vi "Modbus Comm Tester.vi"() -> ()   [LabVIEW 2012]
doc: "Modbus Comm Tester\n\nThis VI demonstrates the usage of the Modbus Master API for both TCP and Serial connections.\nIt is also a useful tool for testing communication with your modbus device. You can test different\ncommunication parameters and coil/register address ranges without having to write any code.\n\nCopyright (c) 2016, Plasmionique Inc.\nAll rights reserved.\n\nLicense: BSD (2-Clause) - http://opensource.org/licenses/BSD-2-Clause"
uses:
  MB_PDU/MB_ReadDevID Codes.ctl
  MB_Master/MB_Master.lvclass
  MB_ADU/MB_ADU.lvclass/MB_ADU.ctl
  MB_ADU/Read TX Data.vi
  MB_ADU/Read RX Data.vi
  MB_ADU/Read RX Timestamp.vi
  MB_Master_Serial/MB_Master_Serial.lvclass
  MB Master.lvlib
  MB_Master_TCP/MB_Master_TCP.lvclass
  MB_ADU/MB_ADU.lvclass
panel:
  in  "Device ID code":T1=1 items=["Basic"=1, "Regular"=2, "Extended"=3, "Single"=4]
  in  "object ID":u8 caption="Object ID"
  in  "Read ID":bool
  out "Open?":bool caption="Connected"
  in  "Tab Control 2":enum32{"Comm Settings", "Comm Status"}(tab)
  in  "Open":bool
  in  "Close":bool
  in  "Type":enum16{"Serial", "TCP"}(ring) caption="Connection Type"
  in  "Tab Control":enum32{"Page 1", "Page 2"}(tab)
  in  "Retries":i32=1
  in  "Timeout (ms)":u32=300
  in  "Flow Control":u16(ring) items=["None", "XON/XOFF", "RTS/CTS", "XON/XOFF & RTS/CTS", "DTR/DSR", "XON/XOFF & DTR/DSR"]
  in  "Parity":u16(ring) items=["None", "Odd", "Even", "Mark", "Space"]
  in  "Stop Bits":u16(ring)=10 items=["1.0"=10, "1.5"=15, "2.0"=20]
  in  "Baud Rate (bps)":u32(ring)=19200 items=["9600"=9600, "19200"=19200, "38400"=38400, "57600"=57600, "115200"=115200, "460800"=460800, "921600"=921600]
  in  "Slave Address":u8=1
  in  "Mode":enum16{"RTU", "ASCII"}(ring)
  in  "COM Port":refnum<visa-resource-name>
  in  "TCP_Port":u16=502 caption="Port"
  in  "IP Address":string="localhost"
  in  "TCP_Timeout":i32=10000 caption="Timeout (ms)"
  in  "TCP_Slave ID":u8=255 caption="Slave ID" format="%.0x"
  in  "Poll Period (ms)":i32=100
  out "Last Error Status":errorcluster
  out "Last RX":string
  out "Last TX":string
  out "Last RX Time":string
  out "Last Error Time":string
  out "dt (ms)":u32
  out "ID objects":string[](array[string]) caption="ID Objects"
  in  "coil Poll":bool
  in  "HR Poll":bool
  in  "DI Poll":bool
  in  "IR Poll":bool
  in  "Write Hld Regs":bool
  in  "Read Hld Regs":bool
  in  "HR QTY":u16=1 caption="Quantity"
  in  "HR SA":u16 caption="Starting Address"
  in  "Holding Registers":u16[](array[numeric])
  in  "Read In Regs":bool
  in  "IR QTY":u16=1 caption="Quantity"
  in  "IR SA":u16 caption="Starting Address"
  out "Input Registers":u16[](array[numeric])
  in  "Read DIs":bool
  in  "DI QTY":u16=1 caption="Quantity"
  in  "DI SA":u16 caption="Starting Address"
  out "Discrete Inputs":bool[](array[boolean])
  in  "Write Coils":bool
  in  "Read Coils":bool
  in  "Coil QTY":u16=1 caption="Quantity"
  in  "Coil SA":u16 caption="Starting Address"
  in  "Coils":bool[](array[boolean])
  # "Input Registers"
  # "Discrete Inputs"
  # "Device ID Objects"
  # "Holding Registers"
  # "Coils"
  # "Communication Settngs"
  # "Communication Status"
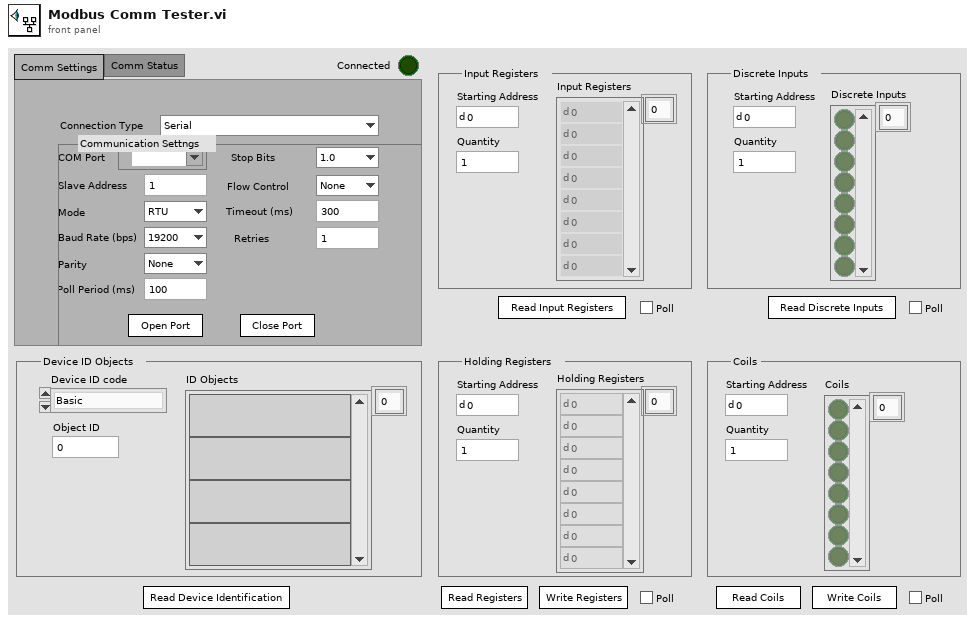
[diagram p1: front panel]
types:
  T1 = typedef "MB Master.lvlib/MB_ReadDevID Codes.ctl" = u8
  T2 = cluster{"baud rate (bps)":u32, "stop bits":u16, "parity":u16, "flow control":u16, "timeout":u32, "retries":i32}
  T3 = typedef "MB Master.lvlib/MB_DevID Object.ctl" = cluster{"ID":u8, "Value":string}
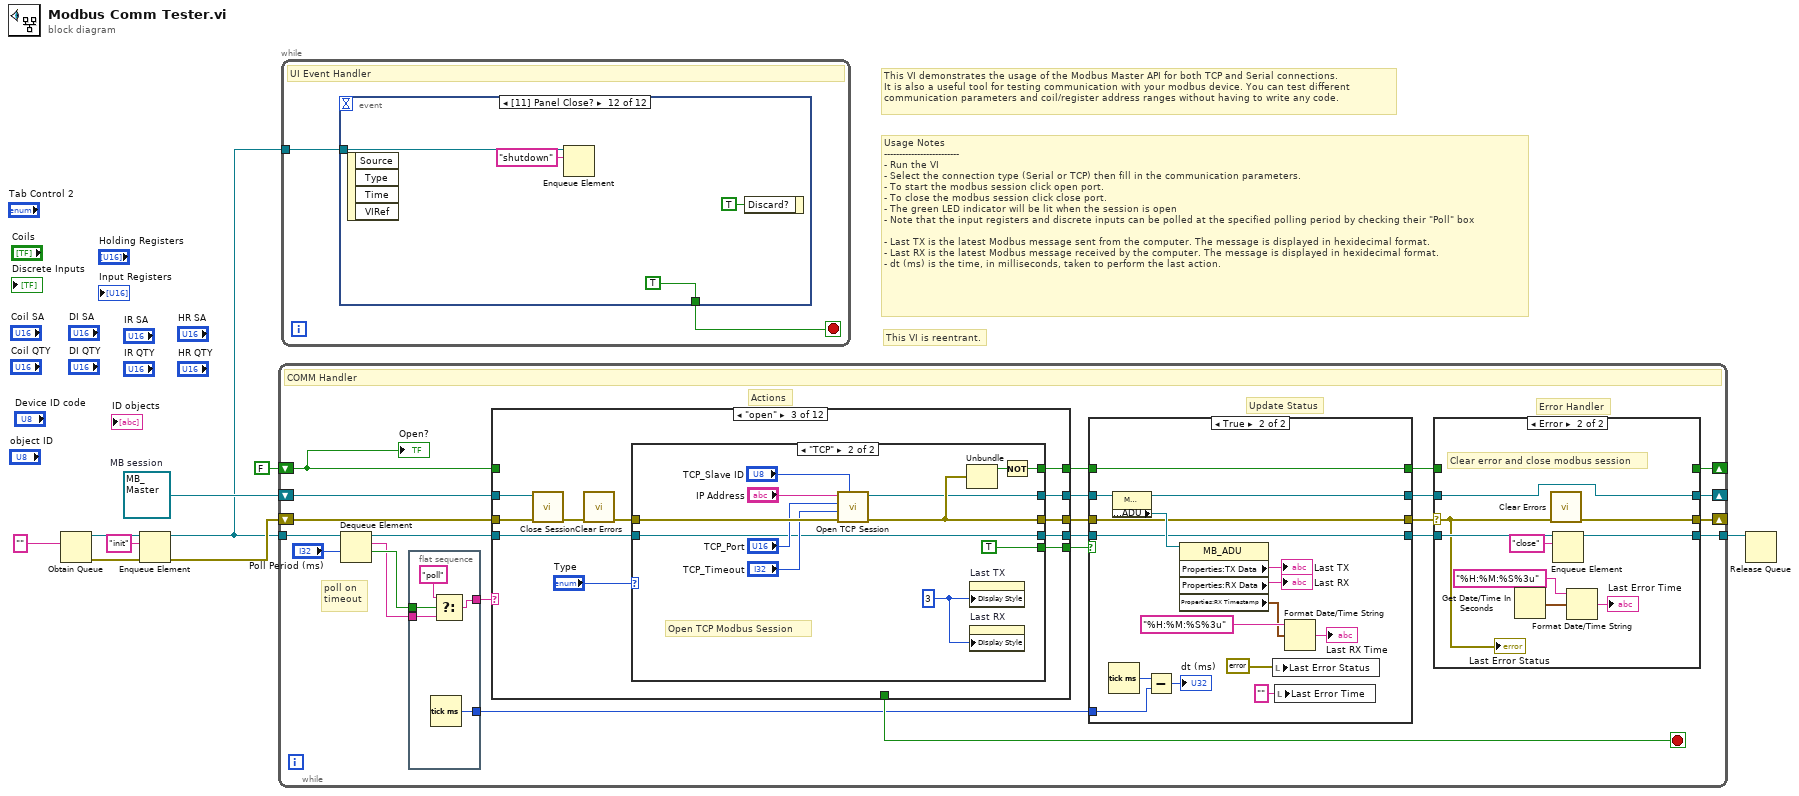
[diagram p0: block diagram]
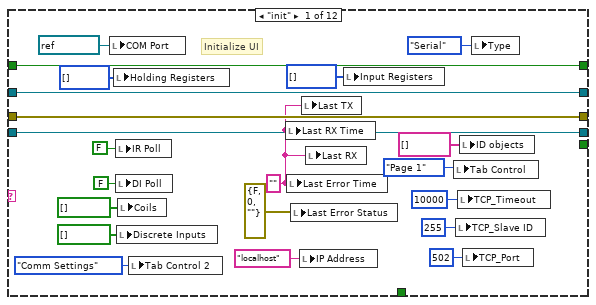
[diagram p4: hidden frame]
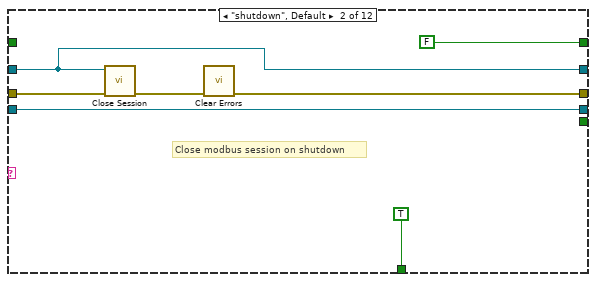
[diagram p5: hidden frame]
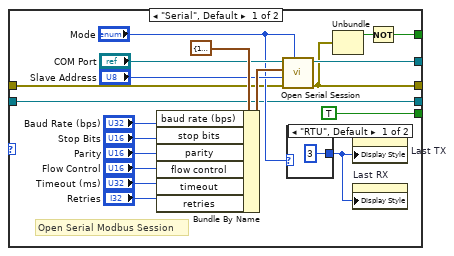
[diagram p6: hidden frame]
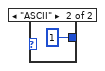
[diagram p7: hidden frame]
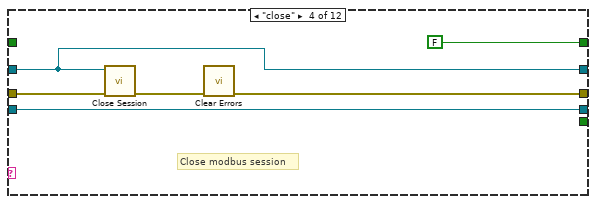
[diagram p8: hidden frame]
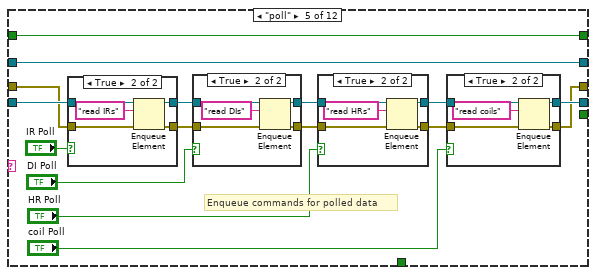
[diagram p9: hidden frame]
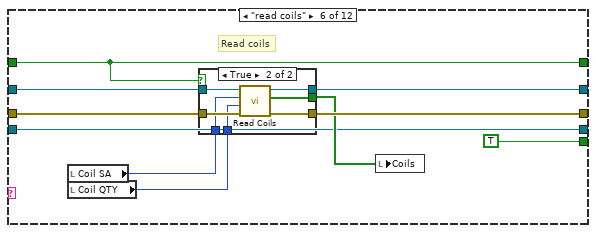
[diagram p14: hidden frame]
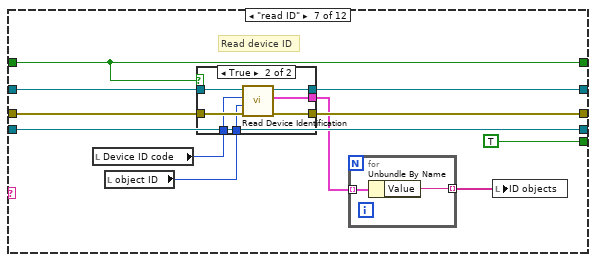
[diagram p16: hidden frame]
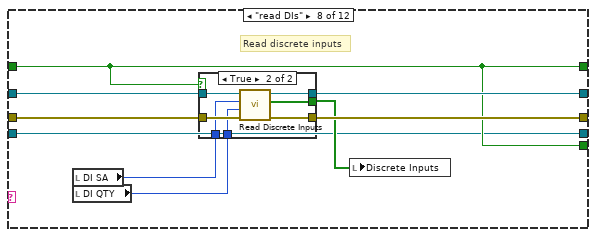
[diagram p18: hidden frame]
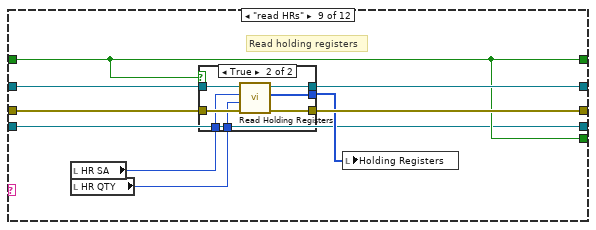
[diagram p20: hidden frame]
diagram:
  w7 = refnum<class "MB_Master.lvclass"> refnum  # MB session
  # "This VI is reentrant."
  # "Usage Notes\n-------------------------\n- Run the VI\n- Select the connection type (Serial or TCP) then fill in the communication parameters.\n- To start the modbus session click open port.\n- To close the modbus session click close port.\n- The green LED indicator will be lit when the session is open\n- Note that the input registers and discrete inputs can be polled at the specified polling period by checking their \"Poll\" box\n\n- Last TX is the latest Modbus message sent from the computer. The message is displayed in hexidecimal format.\n- Last RX is the latest Modbus message received by the computer. The message is displayed in hexidecimal format. \n- dt (ms) is the time, in milliseconds, taken to perform the last action."
  # "This VI demonstrates the usage of the Modbus Master API for both TCP and Serial connections.\nIt is also a useful tool for testing communication with your modbus device. You can test different\ncommunication parameters and coil/register address ranges without having to write any code."
  n1 = Obtain Queue(element data type="") -> (queue out=w6:refnum<queue>, error out=w4:errorcluster)  [unwired: 4 in, 1 out]
  n2 = Enqueue Element(queue=w6, element="init", error in (no error)=w4) -> (queue out=w2:refnum<queue>, error out=w3:errorcluster)  [unwired: 1 in, 1 out]
  n3 = while {
    tunnel: w2 -> [w33]
    shift-right: [w16] -> _
    shift-left: w7 -> [w32]
    shift-right: [w23] -> _
    shift-left: w3 -> [w24]
    shift-right: [w18] -> _
    shift-left: FALSE -> [w28]
    tunnel: [w22] -> w1
    stop <- w31 stop-if-true
    # "poll on\ntimeout"
    # "Actions"
    # "Error Handler"
    # "Update Status"
    # "COMM Handler"
    n4 = Dequeue Element(queue=w33, timeout in ms (-1)="Poll Period (ms)") -> (queue out=w30:refnum<queue>, element=w20:string, timed out?=w21:bool)  [unwired: 1 in, 1 out]
    n5 = flat-sequence {
      tunnel: [w51] -> w25
      tunnel: w21 -> [w50]
      tunnel: w20 -> [w49]
      tunnel: [w47] -> w19
      frame #0 {
        n6 = Tick Count (ms)() -> (millisecond timer value=w51:u32)
        n7 = Select(t="poll", s=w50, f=w49) -> (s? t:f=w47:string)
      }
    }
    n8 = case shown="\"open\"" w19 {
      tunnel: [w91 w96 w110 w146 w158 w201 w221 w241 w259 w277 w297 w331] -> w29
      tunnel: w32 -> [w91 w96 w105 w146 w158 w203 w223 w243 w261 w279 w300 w334]
      tunnel: [w90 w97 w109 w147 w150 w200 w220 w240 w258 w276 w295 w329] -> w13
      tunnel: w24 -> [w90 w99 w104 w149 w162 w202 w222 w242 w260 w278 w296 w330]
      tunnel: [_ TRUE _ _ _ _ _ _ _ _ _ _] -> w31
      tunnel: w30 -> [w81 w93 w101 w144 w164 w194 w217 w235 w253 w271 w289 w323]
      tunnel: w28 -> [w88 _ _ _ w159 w198 w219 w236 w254 w272 w290 w324]
      tunnel: [w88 FALSE w108 FALSE w159 w198 w219 w236 w254 w272 w290 w324] -> w15
      tunnel: [_ _ w107 _ _ TRUE TRUE w236 w254 w272 w290 w324] -> w27
      tunnel: [w81 w93 w100 w144 w156 w194 w217 w235 w253 w271 w289 w323] -> w11
      frame "init" {
        w89 = "" ("Last Error Time")
        # "Initialize UI"
        n9 = local write "COM Port"(refnum<visa-resource-name> refnum ("COM Port")) -> ()
        n10 = local write "Holding Registers"(u16[] [] ("Holding Registers")) -> ()
        n11 = local write "IR Poll"(FALSE ("IR Poll")) -> ()
        n12 = local write "DI Poll"(FALSE ("DI Poll")) -> ()
        n13 = local write "Discrete Inputs"(bool[] [] ("Coils")) -> ()
        n14 = local write "Coils"(bool[] [] ("Coils")) -> ()
        n15 = local write "Tab Control 2"(enum32{"Comm Settings", "Comm Status"}."Comm Settings" ("Tab Control 2")) -> ()
        n16 = local write "Last RX Time"(w89) -> ()
        n17 = local write "Last Error Time"(w89) -> ()
        n18 = local write "Last Error Status"(errorcluster {"status"=FALSE, "code"=0, "source"=""} ("Last Error Status")) -> ()
        n19 = local write "IP Address"("localhost" ("IP Address")) -> ()
        n20 = local write "Last TX"(w89) -> ()
        n21 = local write "Last RX"(w89) -> ()
        n22 = local write "Input Registers"(u16[] [] ("Input Registers")) -> ()
        n23 = local write "Tab Control"(enum32{"Page 1", "Page 2"}."Page 1" ("Tab Control")) -> ()
        n24 = local write "TCP_Slave ID"(u8 255 ("TCP_Slave ID")) -> ()
        n25 = local write "TCP_Timeout"(10000 ("TCP_Timeout")) -> ()
        n26 = local write "ID objects"(string[] [] ("ID objects")) -> ()
        n27 = local write "TCP_Port"(u16 502 ("TCP_Port")) -> ()
        n28 = local write "Type"(enum16{"Serial", "TCP"}."Serial" ("Type")) -> ()
      }
      frame "shutdown", Default {
        # "Close modbus session on shutdown"
        n29 = call-dynamic "Close Session.vi"("error in (no error)"=w99, "MB session in"=w96) -> ("error out"=w98:errorcluster)  [unwired: 9 in]
        n30 = call <vilib>:"Clear Errors.vi"("error in (no error)"=w98) -> ("error out"=w97:errorcluster)  [unwired: 6 in]
      }
      frame "open" {
        n31 = call-dynamic "Close Session.vi"("error in (no error)"=w104, "MB session in"=w105) -> ("error out"=w106:errorcluster)  [unwired: 9 in]
        n32 = call <vilib>:"Clear Errors.vi"("error in (no error)"=w106) -> ("error out"=w103:errorcluster)  [unwired: 6 in]
        n33 = case shown="\"TCP\"" "Type" {
          tunnel: [w119 w132] -> w110
          tunnel: [w118 w133] -> w109
          tunnel: [w116 w136] -> w108
          tunnel: [TRUE TRUE] -> w107
          tunnel: w103 -> [w112 w143]
          tunnel: [w111 w138] -> w100
          tunnel: w101 -> [w111 w138]
          frame "Serial", Default {
            # "Open Serial Modbus Session"
            n34 = Bundle By Name(cluster=T2 {"baud rate (bps)"=19200, "stop bits"=10, "parity"=0, "flow control"=0, "timeout"=1000, "retries"=1} ("Serial Config"), "baud rate (bps)"="Baud Rate (bps)", "stop bits"="Stop Bits", "parity"="Parity", "flow control"="Flow Control", "timeout"="Timeout (ms)", "retries"="Retries") -> (w121:T2)
            n35 = call "Open Serial Session.vi"("Mode (RTU)"="Mode", "Error in"=w112, "Slave ID"="Slave Address", "Serial Config"=w121, "VISA Resource"="COM Port") -> ("Error out"=w118:errorcluster, "MB_Serial session"=w119:refnum<class "MB_Master_Serial.lvclass">)  [unwired: 5 in]
            n36 = case shown="\"RTU\", Default" "Mode" {
              tunnel: [u32 3 ("Display Style") u32 1 ("Display Style")] -> w113
              frame "RTU", Default {
              }
              frame "ASCII" {
              }
            }
            n37 = Unbundle(w118) -> ("status"=w117:bool)  [unwired: 2 out]
            n38 = property on="Last TX" class="Str"("Display Style"=w113) -> ()  [unwired: 2 in, 2 out]
            n39 = property on="Last RX" class="Str"("Display Style"=w113) -> ()  [unwired: 2 in, 2 out]
            n40 = Not(x=w117) -> (.not. x?=w116:bool)
          }
          frame "TCP" {
            w135 = u32 3 ("Display Style")
            # "Open TCP Modbus Session"
            n41 = call "Open TCP Session.vi"("Slave ID (255)"="TCP_Slave ID", "error in (no error)"=w143, "Timeout (10000)"="TCP_Timeout", "Port (502)"="TCP_Port", "IP Address"="IP Address") -> ("error out"=w133:errorcluster, "MB_TCP session"=w132:refnum<class "MB_Master_TCP.lvclass">)  [unwired: 5 in]
            n42 = Unbundle(w133) -> ("status"=w137:bool)  [unwired: 2 out]
            n43 = property on="Last TX" class="Str"("Display Style"=w135) -> ()  [unwired: 2 in, 2 out]
            n44 = property on="Last RX" class="Str"("Display Style"=w135) -> ()  [unwired: 2 in, 2 out]
            n45 = Not(x=w137) -> (.not. x?=w136:bool)
          }
        }
      }
      frame "close" {
        # "Close modbus session"
        n46 = call-dynamic "Close Session.vi"("error in (no error)"=w149, "MB session in"=w146) -> ("error out"=w148:errorcluster)  [unwired: 9 in]
        n47 = call <vilib>:"Clear Errors.vi"("error in (no error)"=w148) -> ("error out"=w147:errorcluster)  [unwired: 6 in]
      }
      frame "poll" {
        # "Enqueue commands for polled data"
        n48 = case shown="True" "IR Poll" {
          tunnel: w164 -> [w188 w192]
          tunnel: [w188 w191] -> w163
          tunnel: w162 -> [w187 w190]
          tunnel: [w187 w189] -> w160
          frame False {
          }
          frame True {
            n49 = Enqueue Element(queue=w192, element="read IRs", error in (no error)=w190) -> (queue out=w191:refnum<queue>, error out=w189:errorcluster)  [unwired: 1 in, 1 out]
          }
        }
        n50 = case shown="True" "DI Poll" {
          tunnel: w163 -> [w180 w185]
          tunnel: w160 -> [w181 w184]
          tunnel: [w181 w183] -> w154
          tunnel: [w180 w182] -> w157
          frame False {
          }
          frame True {
            n51 = Enqueue Element(queue=w185, element="read DIs", error in (no error)=w184) -> (queue out=w182:refnum<queue>, error out=w183:errorcluster)  [unwired: 1 in, 1 out]
          }
        }
        n52 = case shown="True" "HR Poll" {
          tunnel: w157 -> [w173 w178]
          tunnel: w154 -> [w174 w177]
          tunnel: [w174 w176] -> w152
          tunnel: [w173 w175] -> w155
          frame False {
          }
          frame True {
            n53 = Enqueue Element(queue=w178, element="read HRs", error in (no error)=w177) -> (queue out=w175:refnum<queue>, error out=w176:errorcluster)  [unwired: 1 in, 1 out]
          }
        }
        n54 = case shown="True" "coil Poll" {
          tunnel: w155 -> [w166 w171]
          tunnel: w152 -> [w167 w170]
          tunnel: [w167 w169] -> w150
          tunnel: [w166 w168] -> w156
          frame False {
          }
          frame True {
            n55 = Enqueue Element(queue=w171, element="read coils", error in (no error)=w170) -> (queue out=w168:refnum<queue>, error out=w169:errorcluster)  [unwired: 1 in, 1 out]
          }
        }
      }
      frame "read coils" {
        # "Read coils"
        n56 = local read "Coil SA"() -> (w197:u16)
        n57 = local read "Coil QTY"() -> (w196:u16)
        n58 = case shown="True" w198 {
          tunnel: w203 -> [w205 w212]
          tunnel: w202 -> [w204 w211]
          tunnel: [w205 w210] -> w201
          tunnel: [w204 w209] -> w200
          tunnel: w197 -> [_ w208]
          tunnel: w196 -> [_ w207]
          tunnel: [_ w206] -> w199
          frame False {
          }
          frame True {
            n59 = call "Read Coils.vi"("error in (no error)"=w211, "quantity"=w207, "starting address"=w208, "MB session in"=w212) -> ("error out"=w209:errorcluster, "Coils"=w206:bool[], "MB session out"=w210:refnum<class "MB_Master.lvclass">)  [unwired: 5 in]
          }
        }
        n60 = local write "Coils"(w199) -> ()
      }
      frame "read ID" {
        # "Read device ID"
        n61 = local read "Device ID code"() -> (w215:T1)
        n62 = local read "object ID"() -> (w216:u8)
        n63 = case shown="True" w219 {
          tunnel: w223 -> [w227 w232]
          tunnel: w222 -> [w226 w234]
          tunnel: [w227 w231] -> w221
          tunnel: [w226 w233] -> w220
          tunnel: [_ w230] -> w214
          tunnel: w216 -> [_ w229]
          tunnel: w215 -> [_ w228]
          frame False {
          }
          frame True {
            n64 = call "Read Device Identification.vi"("error in (no error)"=w234, "object ID"=w229, "read device ID code"=w228, "MB session in"=w232) -> ("error out"=w233:errorcluster, "DevID Objects"=w230:T3[], "MB session out"=w231:refnum<class "MB_Master.lvclass">)  [unwired: 4 in, 1 out]
          }
        }
        n65 = for {
          tunnel: w214 -> [w225] mode=indexing
          tunnel: [w224] -> w213 mode=indexing
          n66 = Unbundle By Name(w225) -> ("Value"=w224:string)
        }
        n67 = local write "ID objects"(w213) -> ()
      }
      frame "read DIs" {
        # "Read discrete inputs"
        n68 = local read "DI SA"() -> (w238:u16)
        n69 = local read "DI QTY"() -> (w237:u16)
        n70 = case shown="True" w236 {
          tunnel: w243 -> [w245 w252]
          tunnel: w242 -> [w244 w251]
          tunnel: [w245 w250] -> w241
          tunnel: [w244 w249] -> w240
          tunnel: w238 -> [_ w248]
          tunnel: w237 -> [_ w247]
          tunnel: [_ w246] -> w239
          frame False {
          }
          frame True {
            n71 = call "Read Discrete Inputs.vi"("error in (no error)"=w251, "quantity"=w247, "starting address"=w248, "MB session in"=w252) -> ("error out"=w249:errorcluster, "Inputs"=w246:bool[], "MB session out"=w250:refnum<class "MB_Master.lvclass">)  [unwired: 5 in]
          }
        }
        n72 = local write "Discrete Inputs"(w239) -> ()
      }
      frame "read HRs" {
        # "Read holding registers"
        n73 = local read "HR SA"() -> (w256:u16)
        n74 = local read "HR QTY"() -> (w255:u16)
        n75 = case shown="True" w254 {
          tunnel: w261 -> [w263 w270]
          tunnel: w260 -> [w262 w269]
          tunnel: [w263 w268] -> w259
          tunnel: [w262 w267] -> w258
          tunnel: w256 -> [_ w266]
          tunnel: w255 -> [_ w265]
          tunnel: [_ w264] -> w257
          frame False {
          }
          frame True {
            n76 = call "Read Holding Registers.vi"("error in (no error)"=w269, "quantity"=w265, "starting address"=w266, "MB session in"=w270) -> ("error out"=w267:errorcluster, "Registers"=w264:u16[], "MB session out"=w268:refnum<class "MB_Master.lvclass">)  [unwired: 5 in]
          }
        }
        n77 = local write "Holding Registers"(w257) -> ()
      }
      frame "read IRs" {
        # "Read input registers"
        n78 = local read "IR SA"() -> (w274:u16)
        n79 = local read "IR QTY"() -> (w273:u16)
        n80 = case shown="True" w272 {
          tunnel: w279 -> [w281 w288]
          tunnel: w278 -> [w280 w287]
          tunnel: [w281 w286] -> w277
          tunnel: [w280 w285] -> w276
          tunnel: w274 -> [_ w284]
          tunnel: w273 -> [_ w283]
          tunnel: [_ w282] -> w275
          frame False {
          }
          frame True {
            n81 = call "Read Input Registers.vi"("error in (no error)"=w287, "quantity"=w283, "starting address"=w284, "MB session in"=w288) -> ("error out"=w285:errorcluster, "Registers"=w282:u16[], "MB session out"=w286:refnum<class "MB_Master.lvclass">)  [unwired: 5 in]
          }
        }
        n82 = local write "Input Registers"(w275) -> ()
      }
      frame "write coils" {
        # "Write single or multiple coils"
        n83 = local read "Coil SA"() -> (w294:u16)
        n84 = local read "Coil QTY"() -> (w292:u16)
        n85 = local read "Coils"() -> (w293:bool[])
        n86 = Greater?(x=w292, y=u16 1) -> (0:w298:bool)
        n87 = Array Subset(array=w293, length=w292) -> (w291:bool[])  [unwired: 1 in]
        n88 = case shown="True" w290 {
          tunnel: w300 -> [w302 w309]
          tunnel: w298 -> [_ w308]
          tunnel: [w302 w307] -> w297
          tunnel: w296 -> [w301 w306]
          tunnel: [w301 w305] -> w295
          tunnel: w294 -> [_ w304]
          tunnel: w291 -> [_ w303]
          frame False {
          }
          frame True {
            n89 = case shown="True" w308 {
              tunnel: w309 -> [w316 w322]
              tunnel: [w310 w321] -> w307
              tunnel: w306 -> [w315 w320]
              tunnel: [w311 w319] -> w305
              tunnel: w304 -> [w314 w318]
              tunnel: w303 -> [w313 w317]
              frame False {
                n90 = Index Array(array=w313) -> (element=w312:bool)  [unwired: 1 in]
                n91 = call "Write Single Coil.vi"("error in (no error)"=w315, "value"=w312, "address"=w314, "MB session in"=w316) -> ("error out"=w311:errorcluster, "MB session out"=w310:refnum<class "MB_Master.lvclass">)  [unwired: 6 in]
              }
              frame True {
                n92 = call "Write Multiple Coils.vi"("error in (no error)"=w320, "values"=w317, "starting address"=w318, "MB session in"=w322) -> ("error out"=w319:errorcluster, "MB session out"=w321:refnum<class "MB_Master.lvclass">)  [unwired: 6 in]
              }
            }
          }
        }
      }
      frame "write HRs" {
        # "Write single or multiple holding registers"
        n93 = local read "Holding Registers"() -> (w327:u16[])
        n94 = local read "HR SA"() -> (w328:u16)
        n95 = local read "HR QTY"() -> (w326:u16)
        n96 = Greater?(x=w326, y=u16 1) -> (0:w332:bool)
        n97 = Array Subset(array=w327, length=w326) -> (w325:u16[])  [unwired: 1 in]
        n98 = case shown="True" w324 {
          tunnel: w334 -> [w336 w343]
          tunnel: w332 -> [_ w342]
          tunnel: [w336 w341] -> w331
          tunnel: w330 -> [w335 w340]
          tunnel: [w335 w339] -> w329
          tunnel: w328 -> [_ w338]
          tunnel: w325 -> [_ w337]
          frame False {
          }
          frame True {
            n99 = case shown="True" w342 {
              tunnel: w343 -> [w350 w356]
              tunnel: [w344 w355] -> w341
              tunnel: w340 -> [w349 w354]
              tunnel: [w345 w353] -> w339
              tunnel: w338 -> [w348 w352]
              tunnel: w337 -> [w347 w351]
              frame False {
                n100 = Index Array(array=w347) -> (element=w346:u16)  [unwired: 1 in]
                n101 = call "Write Single Register.vi"("error in (no error)"=w349, "value"=w346, "address"=w348, "MB session in"=w350) -> ("error out"=w345:errorcluster, "MB session out"=w344:refnum<class "MB_Master.lvclass">)  [unwired: 6 in]
              }
              frame True {
                n102 = call "Write Multiple Registers.vi"("error in (no error)"=w354, "values"=w351, "starting address"=w352, "MB session in"=w356) -> ("error out"=w353:errorcluster, "MB session out"=w355:refnum<class "MB_Master.lvclass">)  [unwired: 6 in]
              }
            }
          }
        }
      }
    }
    n103 = case shown="True" w27 {
      tunnel: w29 -> [w55 w56]
      tunnel: [w55 w69] -> w17
      tunnel: w25 -> [_ w63]
      tunnel: w15 -> [w54 w59]
      tunnel: [w54 w59] -> w14
      tunnel: w13 -> [w53 w58]
      tunnel: [w53 w58] -> w12
      tunnel: w11 -> [w52 w57]
      tunnel: [w52 w57] -> w10
      frame False {
      }
      frame True {
        n104 = Tick Count (ms)() -> (millisecond timer value=w62:u32)
        n105 = property class="MB_Master"(reference=w56) -> (reference out=w69:refnum<class "MB_Master.lvclass">, "Properties:ADU"=w70:refnum<class "MB_ADU.lvclass">)  [unwired: 1 in, 1 out]
        n106 = Subtract(x=w62, y=w63) -> (x-y=→"dt (ms)":u32)
        n107 = property class="MB_ADU"(reference=w70) -> ("Properties:TX Data"=→"Last TX":string, "Properties:RX Data"=→"Last RX":string, "Properties:RX Timestamp"=w60:timestamp)  [unwired: 1 in, 2 out]
        n108 = local write "Last Error Status"(errorcluster {"status"=FALSE, "code"=0, "source"=""} ("Last Error Status")) -> ()
        n109 = local write "Last Error Time"("" ("Last Error Time")) -> ()
        n110 = Format Date/Time String(time format string (%c)="%H:%M:%S%3u", seconds (now)=w60) -> (date/time string=→"Last RX Time":string)  [unwired: 1 in]
      }
    }
    n111 = case shown="Error" w12 {
      selector: w12 -> [w37 w39]
      tunnel: [w37 w43] -> w23
      tunnel: w10 -> [w36 w41]
      tunnel: [w36 w40] -> w22
      tunnel: w14 -> [w35 _]
      tunnel: [w35 _] -> w18
      tunnel: w17 -> [w34 w38]
      tunnel: [w34 w38] -> w16
      frame No Error {
      }
      frame Error {
        # "Clear error and close modbus session"
        n112 = Get Date/Time In Seconds() -> (seconds since 1Jan1904=w44:timestamp)
        n113 = call <vilib>:"Clear Errors.vi"("error in (no error)"=w39) -> ("error out"=w43:errorcluster)  [unwired: 6 in]
        n114 = Enqueue Element(queue=w41, element="close") -> (queue out=w40:refnum<queue>)  [unwired: 2 in, 2 out]
        n115 = Format Date/Time String(time format string (%c)="%H:%M:%S%3u", seconds (now)=w44) -> (date/time string=→"Last Error Time":string)  [unwired: 1 in]
        "Last Error Status" <- w39
      }
    }
    "Open?" <- w28
  }
  n116 = while {
    tunnel: w2 -> [w358]
    stop <- w357 stop-if-true
    # "UI Event Handler"
    n117 = event shown="[11] Panel Close?" {
      selector: _ -> [_ _ _ _ _ _ _ _ _ _ _ _]
      dyn-events: _ -> [_ _ _ _ _ _ _ _ _ _ _ _]
      timeout: _ -> [_ _ _ _ _ _ _ _ _ _ _ _]
      tunnel: w358 -> [_ w362 w365 w366 w368 w370 w372 w374 w376 w378 w380 w382]
      tunnel: [_ _ _ _ _ _ _ _ _ _ _ TRUE] -> w357
      event Timeout {
        n118 = event-data() -> ()  [unwired: 1 in, 3 out]
      }
      event "Type": Value Change {
        # "Transparent (invisible) tab control contains comm parameter controls"
        # "Change connection type"
        n119 = event-data() -> ("NewVal"=w361:enum16{"Serial", "TCP"})  [unwired: 1 in, 5 out]
        n120 = Type Cast(type="Tab Control", x=w361) -> (*(type *) &x=w359:enum32{"Page 1", "Page 2"})
        n121 = local write "Tab Control"(w359) -> ()
        n122 = Enqueue Element(queue=w362, element="close") -> ()  [unwired: 2 in, 3 out]
      }
      event "Open": Value Change {
        # "Open modbus session"
        n123 = event-data() -> ()  [unwired: 1 in, 6 out]
        n124 = Enqueue Element(queue=w365, element="open") -> ()  [unwired: 2 in, 3 out]
      }
      event "Close": Value Change {
        # "Close modbus session"
        n125 = event-data() -> ()  [unwired: 1 in, 6 out]
        n126 = Enqueue Element(queue=w366, element="close") -> ()  [unwired: 2 in, 3 out]
      }
      event "Read Coils": Value Change {
        n127 = event-data() -> ()  [unwired: 1 in, 6 out]
        n128 = Enqueue Element(queue=w368, element="read coils") -> ()  [unwired: 2 in, 3 out]
      }
      event "Read ID": Value Change {
        n129 = event-data() -> ()  [unwired: 1 in, 6 out]
        n130 = Enqueue Element(queue=w370, element="read ID") -> ()  [unwired: 2 in, 3 out]
      }
      event "Read DIs": Value Change {
        n131 = event-data() -> ()  [unwired: 1 in, 6 out]
        n132 = Enqueue Element(queue=w372, element="read DIs") -> ()  [unwired: 2 in, 3 out]
      }
      event "Write Coils": Value Change {
        n133 = event-data() -> ()  [unwired: 1 in, 6 out]
        n134 = Enqueue Element(queue=w374, element="write coils") -> ()  [unwired: 2 in, 3 out]
      }
      event "Read In Regs": Value Change {
        n135 = event-data() -> ()  [unwired: 1 in, 6 out]
        n136 = Enqueue Element(queue=w376, element="read IRs") -> ()  [unwired: 2 in, 3 out]
      }
      event "Read Hld Regs": Value Change {
        n137 = event-data() -> ()  [unwired: 1 in, 6 out]
        n138 = Enqueue Element(queue=w378, element="read HRs") -> ()  [unwired: 2 in, 3 out]
      }
      event "Write Hld Regs": Value Change {
        n139 = event-data() -> ()  [unwired: 1 in, 6 out]
        n140 = Enqueue Element(queue=w380, element="write HRs") -> ()  [unwired: 2 in, 3 out]
      }
      event Panel Close? {
        n141 = event-data() -> ()  [unwired: 1 in, 4 out]
        n142 = Enqueue Element(queue=w382, element="shutdown") -> ()  [unwired: 2 in, 3 out]
        n143 = event-data("Discard?"=TRUE) -> ()  [unwired: 1 in, 1 out]
      }
    }
  }
  n144 = Release Queue(queue=w1) -> ()  [unwired: 2 in, 3 out]
